vi "Limit Switch Test.vi"() -> ()   [LabVIEW 2025]
uses:
  Libraries/USB IO/Classes/USB-6001/USB-6001.lvclass
  <vilib>/Handler Framework/Handler Framework.lvlib
panel:
  out "High/Low":bool
  out "error out":errorcluster
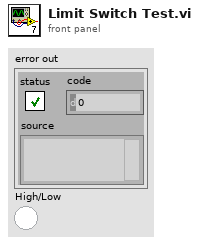
[diagram p1: front panel]
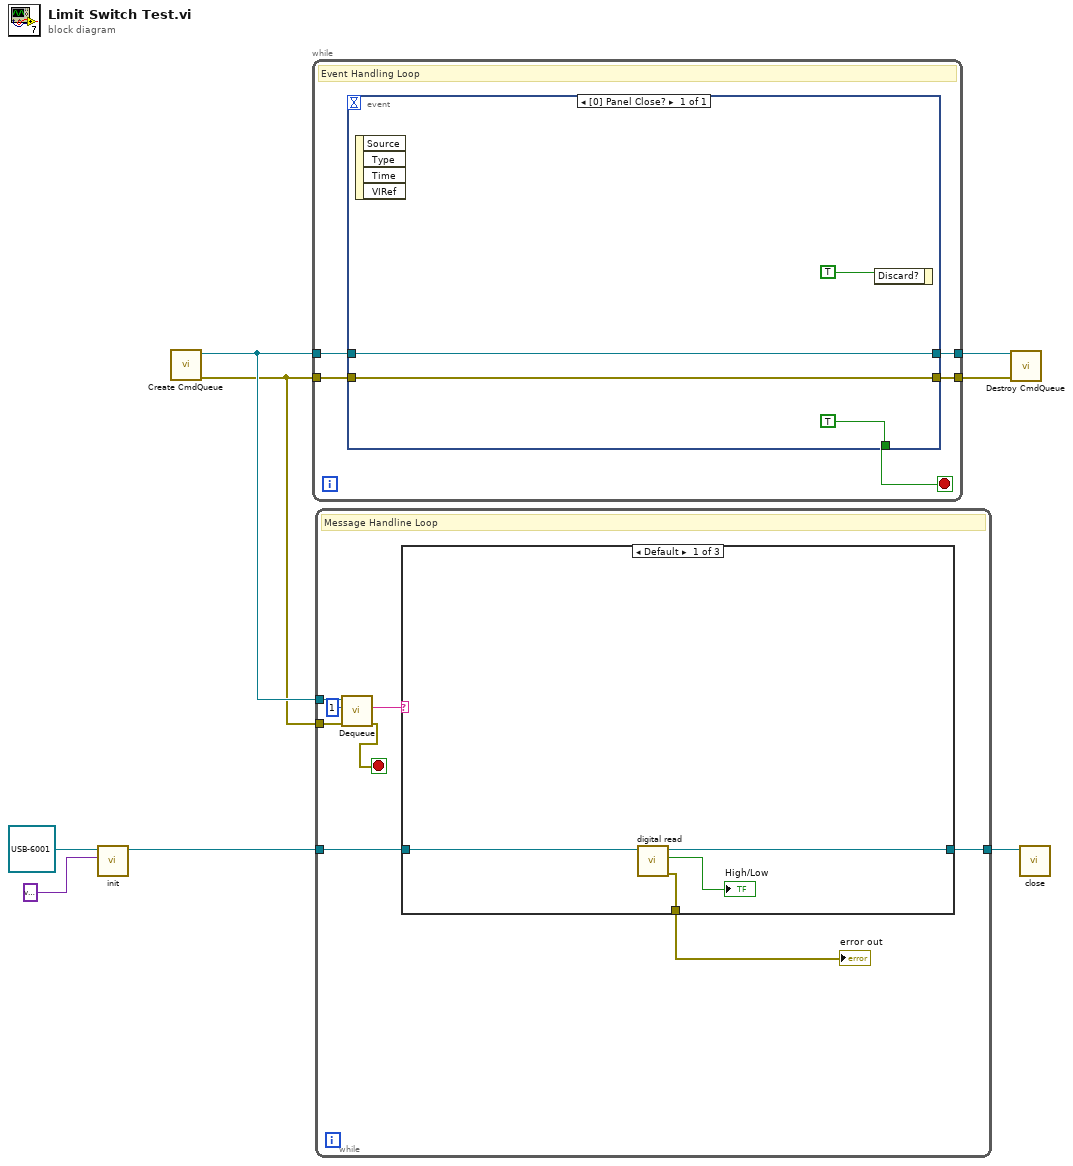
[diagram p0: block diagram]
diagram:
  n1 = call-dynamic "init.vi"("Variant"=variant, "USB-6001 in"=refnum<class "USB-6001.lvclass"> refnum ("USB IO.lvlib:USB-6001.lvclass")) -> ("USB-6001 out"=w2:refnum<class "USB-6001.lvclass">)  [unwired: 8 in, 1 out]
  n2 = call <vilib>:"Create CmdQueue.vi"() -> ("error out"=w7:errorcluster, "CmdQueue out"=w8:refnum<queue>)  [unwired: 10 in]
  n3 = while {
    tunnel: w8 -> [w12]
    tunnel: w7 -> [w11]
    tunnel: [w10] -> w6
    tunnel: [w9] -> w5
    stop <- w13 stop-if-true
    # "Event Handling Loop"
    n4 = event shown="[0] Panel Close?" {
      selector: _ -> [_]
      dyn-events: _ -> [_]
      timeout: _ -> [_]
      tunnel: [TRUE] -> w13
      tunnel: w12 -> [w15]
      tunnel: w11 -> [w14]
      tunnel: [w15] -> w10
      tunnel: [w14] -> w9
      event Panel Close? {
        n5 = event-data() -> ()  [unwired: 1 in, 4 out]
        n6 = event-data("Discard?"=TRUE) -> ()  [unwired: 1 in, 1 out]
      }
    }
  }
  n7 = while {
    tunnel: w8 -> [w25]
    tunnel: w7 -> [w24]
    tunnel: w2 -> [w21]
    tunnel: [w20] -> w1
    stop <- w23 stop-if-true
    # "Message Handline Loop"
    n8 = call <vilib>:"Dequeue.vi"("error in (no error)"=w24, "timeout in ms (-1)"=1, "CmdQueue in"=w25) -> ("error out"=w23:errorcluster, "cmd"=w22:string)  [unwired: 4 in, 3 out]
    n9 = case shown="Default" w22 {
      tunnel: w21 -> [w29 w30 w31]
      tunnel: [w28 w30 w31] -> w20
      tunnel: [w27 _ _] -> w18
      frame Default {
        n10 = call-dynamic "digital read.vi"("USB-6001 in"=w29) -> ("error out"=w27:errorcluster, "High/Low"=→"High/Low":bool, "USB-6001 out"=w28:refnum<class "USB-6001.lvclass">)  [unwired: 8 in]
      }
      frame "init" {
      }
      frame "shutdown" {
      }
    }
    "error out" <- w18
  }
  n11 = call <vilib>:"Destroy CmdQueue.vi"("error in (no error)"=w5, "CmdQueue in"=w6) -> ()  [unwired: 9 in, 1 out]
  n12 = call-dynamic "close.vi"("USB-6001 in"=w1) -> ()  [unwired: 9 in, 2 out]
